vi "clock_nanosleep.vi"(8 "error in (no error)":errorcluster, 9 "flags":T1, 10 "clockid_t":T2=enum."Monotonic", 11 "request":cluster{"sec":u64, "nsec":u64}) -> (0 "error out":errorcluster, 3 "remain":cluster{"sec":u64, "nsec":u64})   [LabVIEW 2013, in "Linux RT Utilities.lvlib"]
doc: "Wrapper VI for glibc's clock_nanosleep() function."
uses:
  Linux RT Utilities.lvlib
  Controls/Public/C Enums/clockid_t.ctl
  Controls/Public/nanosleep flags.ctl
  <vilib>/Utility/error.llb/Error Cluster From Error Code.vi
  <vilib>/NI/NI Linux RT Errno/VIs/Public/Get LV Error Info from Errno.vi
  <vilib>/NI/NI Linux RT Errno/Linux Errno.lvlib
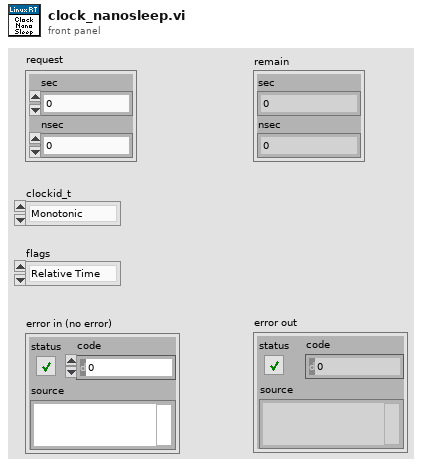
[diagram p1: front panel]
types:
  T1 = typedef "Linux RT Utilities.lvlib/nanosleep flags.ctl" = enum16{"Relative Time", "Absolute Time"}
  T2 = typedef "Linux RT Utilities.lvlib/clockid_t.ctl" = enum16{"Realtime", "Monotonic"}
  T3 = typedef "Linux Errno.lvlib/errno.ctl" = enum16{"NO ERROR", "EPERM", "ENOENT", "ESRCH", "EINTR", "EIO", "ENXIO", "E2BIG", "ENOEXEC", "EBADF", "ECHILD", "EAGAIN", "ENOMEM", "EACCES", "EFAULT", "ENOTBLK", "EBUSY", "EEXIST", "EXDEV", "ENODEV", "ENOTDIR", "EISDIR", "EINVAL", "ENFILE", "EMFILE", "ENOTTY", "ETXTBSY", "EFBIG", "ENOSPC", "ESPIPE", "EROFS", "EMLINK", "EPIPE", "EDOM", "ERANGE", "EDADLK", "ENAMETOOLONG", "ENOLCK", "ENOSYS", "ENOTEMPTY", "ELOOP", "EWOULDBLOCK", "ENOMSG", "EIDRM", "ECHRNG", "EL2NSYNC", "EL3HLT", "EL3RST", "ELNRNG", "EUNATCH", "ENOCSI", "EL2HLT", "EBADE", "EBADR", "EXFULL", "ENOANO", "EBADRQC", "EBADSLT", "EDEADLOCK", "EBFONT", "ENOSTR", "ENODATA", "ETIME", "ENOSR", "ENONET", "ENOPKG", "EREMOTE", "ENOLINK", "EADV", "ESRMNT", "ECOMM", "EPROTO", "EMULTIHOP", "EDOTDOT", "EBADMSG", "EOVERFLOW", "ENOTUNIQ", "EBADFD", "EREMCHG", "ELIBACC", "ELIBBAD", "ELIBSCN", "ELIBMAX", "ELIBEXEC", "ELISEQ", "ERESTART", "ESTRPIPE", "EUSERS", "ENOTSOCK", "EDESTADDRREQ", "EMSGSIZE", "EPROTOTYPE", "ENOPROTOOPT", "EPROTONOSUPPORT", "ESOCKTNOSUPPORT", "EOPNOTSUPP", "EPFNOSUPPORT", "EAFNOSUPPORT", "EADDRINUSE", "EADDRNOTAVAIL", "ENETDOWN", "ENETUNREACH", "ENETRESET", "ECONNABORTED", "ECONNRESET", "ENOBUFS", "EISCONN", "ENOTCONN", "ESHUTDOWN", "ETOOMANYREFS", "ETIMEDOUT", "ECONNREFUSED", "EHOSTDOWN", "EHOSTUNREACH", "EALREADY", "EINPROGRESS", "ESTALE", "EUCLEAN", "ENOTNAM", "ENAVAIL", "EISNAM", "EREMOTEIO", "EDQUOT", "ENOMEDIUM", "EMEDIUMTYPE", "ECANCELED", "ENOKEY", "EKEYEXPIRED", "EKEYREVOKED", "EKEYREJECTED", "EOWNERDEAD", "ENOTRECOVERABLE", "ERFKILL", "EHWPOISON", "UNDEFINED"}
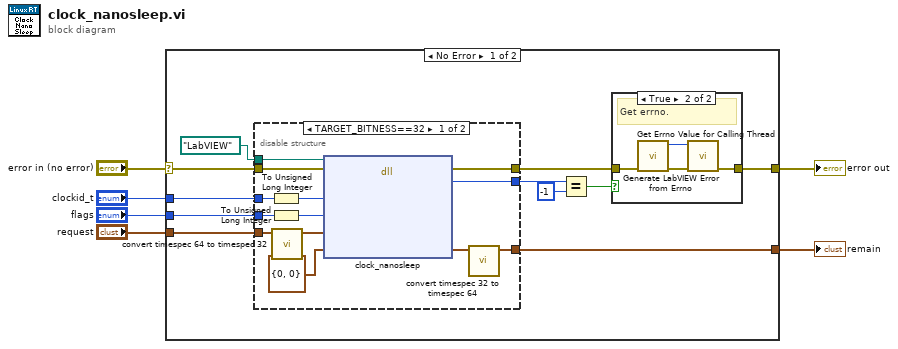
[diagram p0: block diagram]
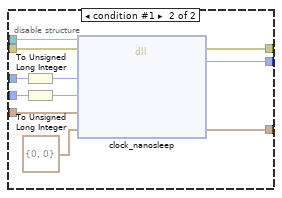
[diagram p3: hidden frame]
diagram:
  n1 = case shown="No Error" "error in (no error)" {
    selector: "error in (no error)" -> [w8 w47]
    tunnel: [w9 w47] -> w5
    tunnel: "request" -> [w15 _]
    tunnel: "clockid_t" -> [w17 _]
    tunnel: "flags" -> [w16 _]
    tunnel: [w14 _] -> w1
    frame No Error {
      n2 = disable-structure shown="TARGET_BITNESS==32" {
        disable-tunnel: [w35 w46] -> w11
        disable-tunnel: w17 -> [w34 w45]
        disable-tunnel: w16 -> [w33 w44]
        disable-tunnel: w15 -> [w28 w37]
        disable-tunnel: w8 -> [w27 w40]
        disable-tunnel: path "LabVIEW" ("Path") -> [w26 w39]
        disable-tunnel: [w24 w38] -> w14
        disable-tunnel: [w23 w36] -> w12
        frame condition #0 (active) {
          n3 = To Unsigned Long Integer(number=w34) -> (unsigned 32bit integer=w32:u32)
          n4 = To Unsigned Long Integer(number=w33) -> (unsigned 32bit integer=w31:u32)
          n5 = call "convert timespec 64 to timespec 32.vi"("timespec 64"=w28) -> ("timespec 32"=w29:cluster{"sec":u32, "nsec":u32})  [unwired: 10 in]
          n6 = dll-call lib="?" fn="clock_nanosleep"(path in=w26, error in=w27, "clockid_t"=w32, "flags"=w31, "request"=w29, "remain"=cluster{"sec":u32, "nsec":u32} {"sec"=0, "nsec"=0} ("timespec")) -> (error out=w35:errorcluster, "status"=w23:i32, "remain"=w25:cluster{"sec":u32, "nsec":u32})  [unwired: 4 in, 1 out]
          n7 = call "convert timespec 32 to timespec 64.vi"("timespec 32"=w25) -> ("timespec 64"=w24:cluster{"sec":u64, "nsec":u64})  [unwired: 10 in]
        }
        frame condition #1 {
          n8 = To Unsigned Long Integer(number=w45) -> (unsigned 32bit integer=w43:u32)
          n9 = To Unsigned Long Integer(number=w44) -> (unsigned 32bit integer=w42:u32)
          n10 = dll-call lib="?" fn="clock_nanosleep"(path in=w39, error in=w40, "clockid_t"=w43, "flags"=w42, "request"=w37, "remain"=cluster{"sec":u64, "nsec":u64} {"sec"=0, "nsec"=0} ("timespec")) -> (error out=w46:errorcluster, "status"=w36:i32, "remain"=w38:cluster{"sec":u64, "nsec":u64})  [unwired: 4 in, 1 out]
        }
      }
      n11 = Equal?(x=w12, y=-1) -> (x = y?=w10:bool)
      n12 = case shown="True" w10 {
        tunnel: w11 -> [w18 w22]
        tunnel: [w18 w19] -> w9
        frame False {
          # "No error."
        }
        frame True {
          # "Get errno."
          n13 = call <vilib>:"Get Errno Value for Calling Thread.vi"("error in (no error)"=w22) -> ("error out"=w21:errorcluster, "errno"=w20:T3)  [unwired: 9 in]
          n14 = call <vilib>:"Generate LabVIEW Error from Errno.vi"("error in (no error)"=w21, "errno"=w20) -> ("error out"=w19:errorcluster)  [unwired: 9 in]
        }
      }
    }
    frame Error {
    }
  }
  "error out" <- w5
  "remain" <- w1
